vi "Finalize.vi"(8 "error in":errorcluster, 11 "Logging Execution Unit in":refnum<class "Logging Execution Unit.lvclass">) -> (0 "error out":errorcluster, 3 "Logging Execution Unit out":refnum<class "Logging Execution Unit.lvclass">)   [LabVIEW 2020, in "AIM ARINC 429 Engine.lvlib" / "Implementation.lvlib" / "Logging Execution Unit.lvclass"]
uses:
  Logging Execution Unit.lvclass
  Logging Execution Unit.lvclass/Logging Execution Unit.ctl
  <vilib>/NI/VeriStand Custom Device Messaging/Message/Shutdown Message/Shutdown Message.lvclass
  C:/Program Files (x86)/National Instruments/LabVIEW 2020/vi.lib/NI/VeriStand Custom Device Messaging/Message/Abstract Message/Abstract Message.lvclass
  Logging/Word Logging/Log Producer/Log Producer.lvclass
  C:/Program Files (x86)/National Instruments/LabVIEW 2020/vi.lib/NI/VeriStand Custom Device Messaging/Producer/Abstract Producer/Abstract Producer.lvclass
  <vilib>/NI/VeriStand Custom Device Messaging/Producer/Abstract Producer/Shutdown.vi
  Logging/Word Logging/Word Logging.lvlib
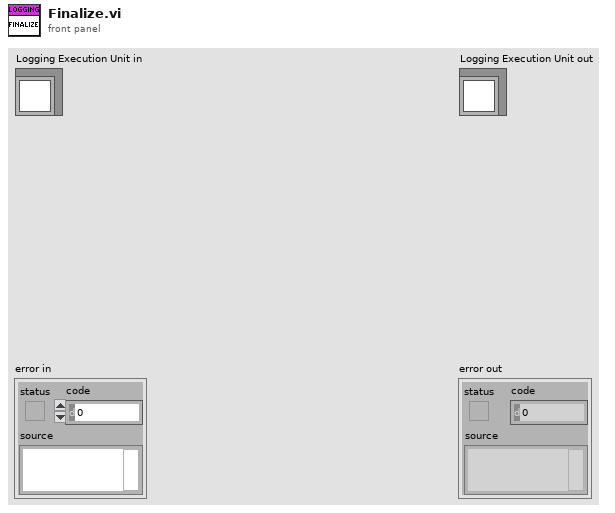
[diagram p1: front panel]
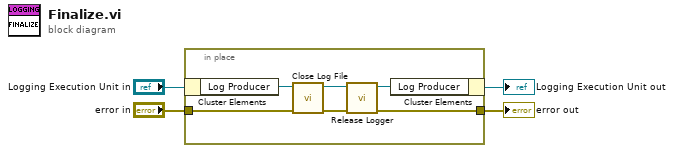
[diagram p0: block diagram]
diagram:
  n1 = in-place {
    in-place-border: [w7] -> w3
    in-place-border: "error in" -> [w5]
    n2 = in-place-cluster #1("Logging Execution Unit in") -> ("Log Producer"=w10:refnum<class "Log Producer.lvclass">)
    n3 = call "Close Log File.vi"("error in (no error)"=w5, "Log Producer in"=w10) -> ("error out"=w8:errorcluster, "Log Producer out"=w9:refnum<class "Log Producer.lvclass">)  [unwired: 8 in]
    n4 = call "Release Logger.vi"("error in (no error)"=w8, "Producer"=w9) -> ("error out"=w7:errorcluster, "Default Producer"=w6:refnum<class "Log Producer.lvclass">)  [unwired: 8 in]
    n5 = in-place-cluster #1("Log Producer"=w6) -> (→"Logging Execution Unit out":refnum<class "Logging Execution Unit.lvclass">)
  }
  "error out" <- w3
